vi "Set Buttons from Objects.vi"(0 "Display State In":T1={"Buttons Displayed"=0, "Button States"=[], "Button Size"=0, "Button Style"=enum."Classic", "Active Button"=0, "Force Regen?"=FALSE, "Tip String Ref"=refnum}, 1 "Lazy Load?":bool=TRUE, 5 "Buttons":refnum<class "Button.lvclass">[](array[class]), 7 "Insert (F=Replace)":bool, 9 "Container State":T3, 11 "error in (no error)":errorcluster, 12 "Index":i32) -> (4 "Display State Out":T1={"Buttons Displayed"=0, "Button States"=[], "Button Size"=0, "Button Style"=enum."Classic", "Active Button"=0, "Force Regen?"=FALSE, "Tip String Ref"=refnum}, 15 "error out":errorcluster)   [LabVIEW 2012, in "Toolbar.xctl"]
doc: "Set lots of buttons from an array of button class objects in one go."
uses:
  Toolbar.xctl
  <vilib>/_xctls/Container State.ctl
  Toolbar State.ctl
  Button_Class/Button.lvclass
  Button_Class/Type Defs/Button Style.ctl
  <vilib>/_xctls/XControlSupport.lvlib
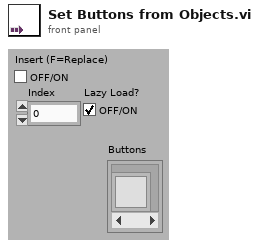
[diagram p1: front panel]
types:
  T1 = typedef "Toolbar.xctl/Toolbar State.ctl" = cluster{"Buttons Displayed":i32, "Button States":refnum<class "Button.lvclass">[], "Button Size":i32, "Button Style":T2, "Active Button":i32, "Force Regen?":bool, "Tip String Ref":refnum<vi>}
  T2 = typedef "Button.lvclass/Button Style.ctl" = enum16{"System", "Modern", "Classic", "Rounded", "Silver", "Ni Theme", "Metallic"}
  T3 = typedef "XControlSupport.lvlib/Container State.ctl" = cluster{"Indicator?":bool, "Run Mode?":bool, " Refnum":refnum<vi>}
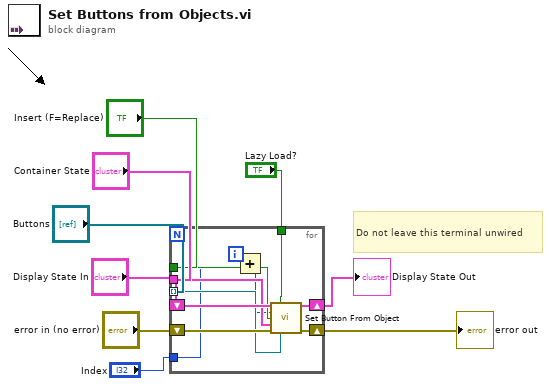
[diagram p0: block diagram]
diagram:
  # "Do not leave this terminal unwired"
  n1 = for {
    shift-right: [w19] -> w3
    shift-left: "Display State In" -> [w20]
    shift-right: [w17] -> w7
    shift-left: "error in (no error)" -> [w18]
    tunnel: "Buttons" -> [w16] mode=indexing
    tunnel: "Container State" -> [w15]
    tunnel: "Insert (F=Replace)" -> [w14]
    tunnel: "Index" -> [w11]
    tunnel: "Lazy Load?" -> [w10]
    i -> [w13]
    n2 = Add(x=w13, y=w11) -> (x+y=w12:i32)
    n3 = call "Set Button From Object.vi"("Display State In"=w20, "Lazy Load?"=w10, "Index (-1=at end)"=w12, "Insert (F=Replace)"=w14, "Container State"=w15, "error in (no error)"=w18, "Button.lvclass"=w16) -> ("Display State Out"=w19:T1, "error out"=w17:errorcluster)  [unwired: 7 out]
  }
  "Display State Out" <- w3
  "error out" <- w7
